vi "Utility - Configuration File Generator.vi"() -> ()   [LabVIEW 2016]
uses:
  <vilib>/LabVIEW Targets/FPGA/cRIO/shared/nicrio_ModuleControls/nicrio_cRIO-9239_DataRatesRing.ctl
  controls/TDMS Properties.ctl
  controls/Acquisition and Logging Configuration.ctl
  <vilib>/Utility/xml.llb/Write to XML File(string).vi
  <vilib>/WebDAVClient/Simple Put File.vi
  <vilib>/WebDAVClient/NI_WebDAV.lvlib
panel:
  in  "Amplitude (0~10) - Vp":dbl=10.0 min=-10.0 max=10.0
  in  "Frequency - Hz":i32=500
  out "Error out WebDAV Put @ cRIO":errorcluster
  in  "TDMS Properties":T1[](array[typedef])=[{"Name"="LIOc/CSUB Soft", "Value"="Teste0112"}, {"Name"="Author", "Value"="[DeveloperName]"}, {"Name"="Operator", "Value"="[OperatorName]"}, {"Name"="TestSystem", "Value"="[SystemName]"}, {"Name"="Site", "Value"="[Location]"}, {"Name"="Line", "Value"="[Line]"}, {"Name"="Machine", "Value"="[MachineName]"}, {"Name"="Description", "Value"="[Description]"}]
  in  "Trigger - Time (Minute)":i32=1
  in  "Trigger - Channel":i32=1
  in  "Trigger - RMS Value":dbl=1.8
  in  "Channel Names":string[](array[string])=["Ch0", "Ch1", "Ch2", "Ch3", "Ch4", "Ch5", "Ch6", "Ch7", "Ch8", "Ch9", "Ch10", "Ch11", "Ch12", "Ch13", "Ch14", "Ch15"]
  in  "Channel Scale Array":fxp<+,24,12>[](array[numeric])=[1.0, 1.0, 1.0, 1.0, 1.0, 1.0, 1.0, 1.0, 1.0, 1.0, 1.0, 1.0, 1.0, 1.0, 1.0, 1.0]
  in  "Number of Channels":i32=16
  in  "Data File Name":string="cRIO_Data_4x239"
  in  "Number of Reads to Save":i32=20
  in  "Samples per Read":i32=12800
  in  "Data Rate":T2=1 items=["50.000 kS/s (NI 9239)"=1, "25.000 kS/s (NI 9239)"=2, "16.667 kS/s (NI 9239)"=3, "12.500 kS/s (NI 9239)"=4, "10.000 kS/s (NI 9239)"=5, "8.333 kS/s (NI 9239)"=6, "7.143 kS/s (NI 9239)"=7, "6.250 kS/s (NI 9239)"=8, "5.556 kS/s (NI 9239)"=9, "5.000 kS/s (NI 9239)"=10, "4.545 kS/s (NI 9239)"=11, "4.167 kS/s (NI 9239)"=12, "3.846 kS/s (NI 9239)"=13, "3.571 kS/s (NI 9239)"=14, "3.333 kS/s (NI 9239)"=15, "3.125 kS/s (NI 9239)"=16, "2.941 kS/s (NI 9239)"=17, "2.778 kS/s (NI 9239)"=18, "2.632 kS/s (NI 9239)"=19, "2.500 kS/s (NI 9239)"=20, "2.381 kS/s (NI 9239)"=21, "2.273 kS/s (NI 9239)"=22, "2.174 kS/s (NI 9239)"=23, "2.083 kS/s (NI 9239)"=24, "2.000 kS/s (NI 9239)"=25, "1.923 kS/s (NI 9239)"=26, "1.852 kS/s (NI 9239)"=27, "1.786 kS/s (NI 9239)"=28, "1.724 kS/s (NI 9239)"=29, "1.667 kS/s (NI 9239)"=30, "1.613 kS/s (NI 9239)"=31]
  # "Gera o arquivo de configuração, em extensão xml, que será lido pela VI \"Get Configuration Settings.vi\"\n na pasta do projeto \"Support VIs\" que se encontra anexada ao target cRIO.\n Informações sobre as funcionalidades adicionadas no diagrama de blocos"
  # "Instructions: Populate the controls below with desired values, then run the VI to generate a 'Config.xml' file in the root folder of your project.  \n\nNote:  Once you have generated the Config.xml file, you will need to copy it to the root folder of your RT Target."
  # "Acquisition"
  # "Channels"
  # "Logging"
  # "Trigger"
  # "Transmission"
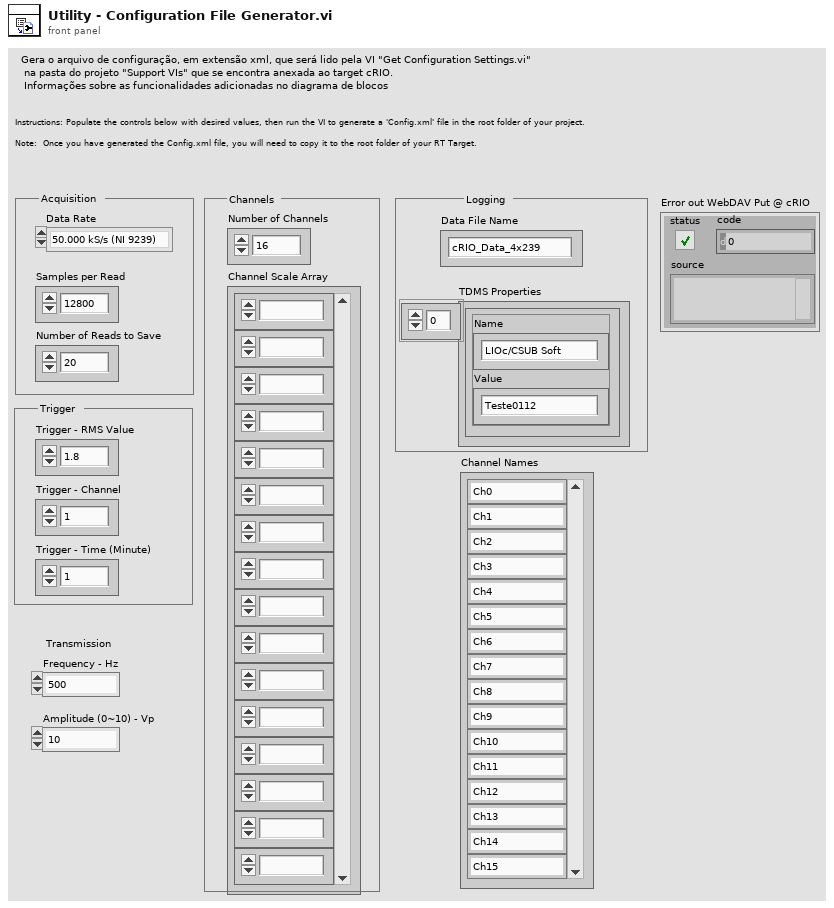
[diagram p1: front panel]
types:
  T1 = typedef "TDMS Properties.ctl" = cluster{"Name":string, "Value":string}
  T2 = typedef "nicrio_cRIO-9239_DataRatesRing.ctl" = u8
  T3 = typedef "Acquisition and Logging Configuration.ctl" = cluster{"Data Rate":T2, "Samples per Read":i32, "Number of Reads to Save":i32, "Data File Name":string, "TDMS Properties":T1[], "Number of Channels":i32, "Channel Scale Array":fxp<+,24,12>[], "Channel Names":string[], "Trigger - RMS Value":dbl, "Trigger - Channel":i32, "Trigger - Time (Minute)":i32, "Frequency ":i32, "Amplitude (0~10)":dbl}
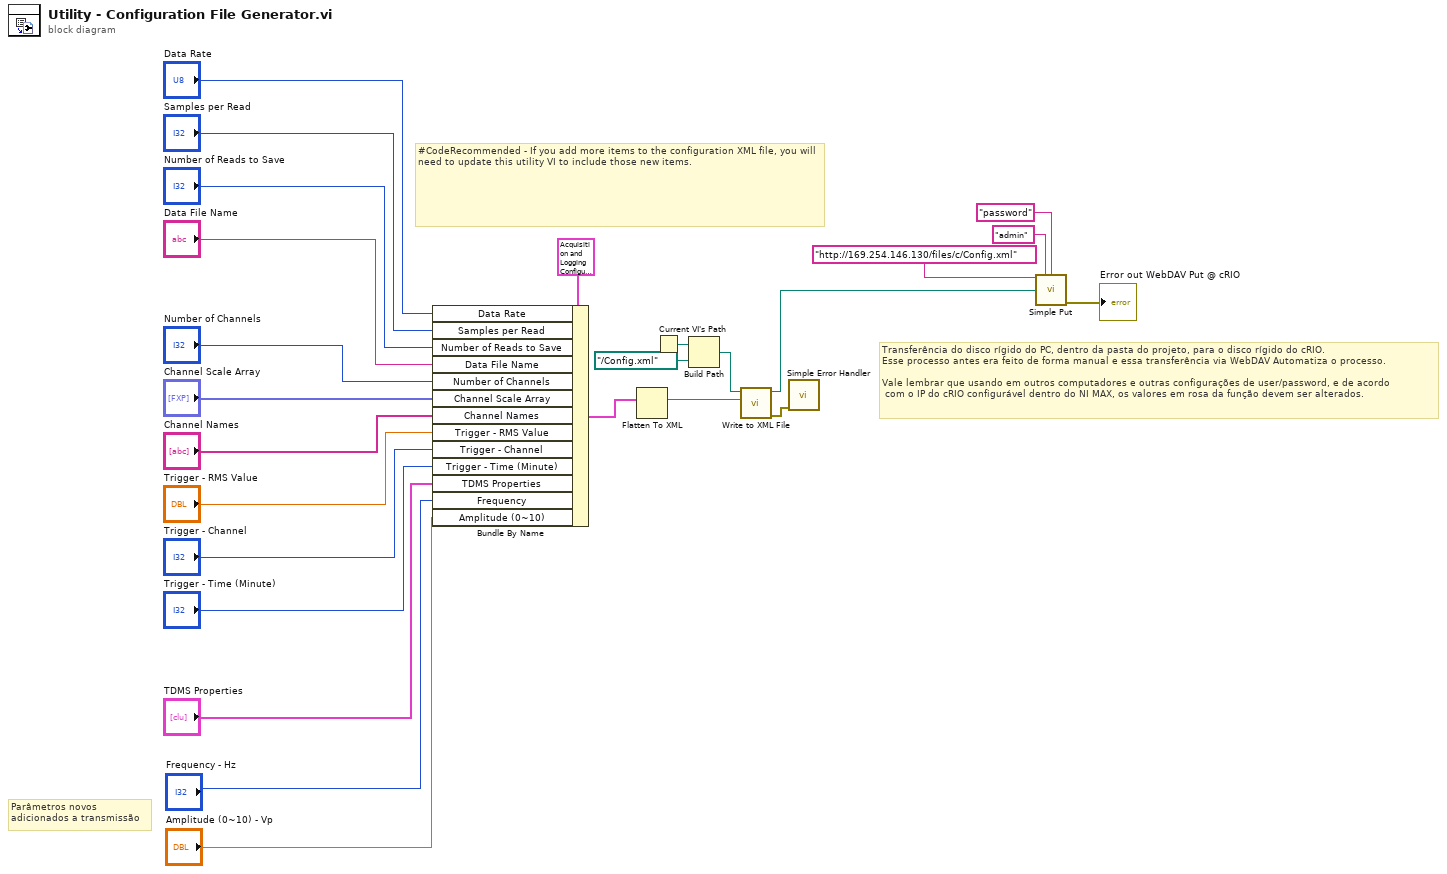
[diagram p0: block diagram]
diagram:
  # "Parâmetros novos \nadicionados a transmissão"
  # "Transferência do disco rígido do PC, dentro da pasta do projeto, para o disco rígido do cRIO.\nEsse processo antes era feito de forma manual e essa transferência via WebDAV Automatiza o processo.\n\nVale lembrar que usando em outros computadores e outras configurações de user/password, e de acordo\n com o IP do cRIO configurável dentro do NI MAX, os valores em rosa da função devem ser alterados."
  # "#CodeRecommended - If you add more items to the configuration XML file, you will need to update this utility VI to include those new items."
  n1 = Bundle By Name(cluster=T3 {"Data Rate"=1, "Samples per Read"=0, "Number of Reads to Save"=0, "Data File Name"="", "TDMS Properties"=[], "Number of Channels"=0, "Channel Scale Array"=[0.0, 0.0, 0.0, 0.0, 1.0, 1.0, 1.0, 1.0, 1.0, 1.0, 1.0, 1.0, 1.0, 1.0, 1.0, 1.0], "Channel Names"=[], "Trigger - RMS Value"=0.0, "Trigger - Channel"=0, "Trigger - Time (Minute)"=0, "Frequency "=0, "Amplitude (0~10)"=0.0} ("Acquisition and Logging Configuration"), "Data Rate"="Data Rate", "Samples per Read"="Samples per Read", "Number of Reads to Save"="Number of Reads to Save", "Data File Name"="Data File Name", "Number of Channels"="Number of Channels", "Channel Scale Array"="Channel Scale Array", "Channel Names"="Channel Names", "Trigger - RMS Value"="Trigger - RMS Value", "Trigger - Channel"="Trigger - Channel", "Trigger - Time (Minute)"="Trigger - Time (Minute)", "TDMS Properties"="TDMS Properties", "Frequency"="Frequency - Hz", "Amplitude (0~10)"="Amplitude (0~10) - Vp") -> (w24:T3)
  n2 = Flatten To XML(anything=w24) -> (xml string=w23:string)
  n3 = Current VI's Path() -> (path=w22:path)
  n4 = Build Path(base path=w22, name or relative path=path "../Config.xml") -> (appended path=w20:path)
  n5 = call-poly <vilib>:"Write to XML File.vi"("XML Input"=w23, "XML File Path"=w20) -> ("error out"=w19:errorcluster, "XML File Path(duplicate)"=w3:path)  [unwired: 7 in, 1 out]
  n6 = call <vilib>:"Simple Error Handler.vi"("error in (no error)"=w19) -> ()  [unwired: 4 in, 5 out]
  n7 = call-poly <vilib>:"Simple Put.vi"("file uri"="http://169.254.146.130/files/c/Config.xml", "username"="admin", "password"="password", "local file path"=w3) -> ("error out"=→"Error out WebDAV Put @ cRIO":errorcluster)  [unwired: 10 in, 1 out]
